vi "Deserialize Connections in Wrapper - Multiple Converter.vi"(11 "error in":errorcluster) -> (15 "error out":errorcluster)   [LabVIEW 2021, in "Converter.lvlib"]
uses:
  Converter.lvlib
  <vilib>/Utility/traverseref.llb/TRef TravTarget.ctl
  <vilib>/Utility/miscctls.llb/LVPointTypeDef.ctl
  <vilib>/Utility/traverseref.llb/VI Scripting - Traverse.lvlib
  Converter Reusables/Converter Reusables.lvlib
  Path Functions/Path Functions.lvlib
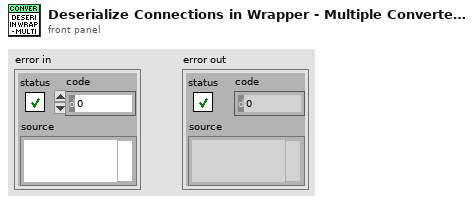
[diagram p1: front panel]
types:
  T1 = typedef "TRef TravTarget.ctl" = enum16{"FP", "BD", "Other"}
  T2 = typedef "LVPointTypeDef.ctl" = cluster{"Horizontal":i16, "Vertical":i16}
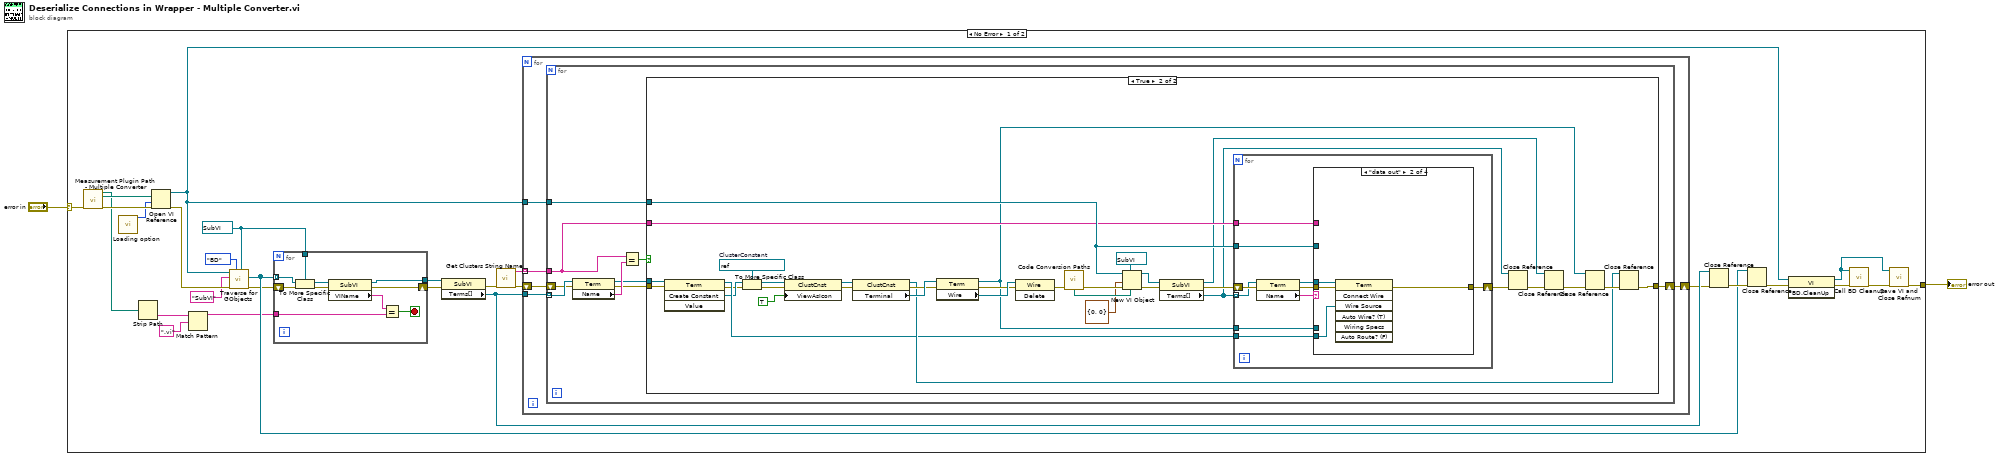
[diagram p0: block diagram]
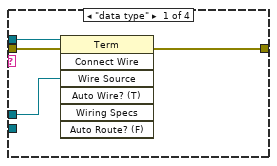
[diagram p3: hidden frame]
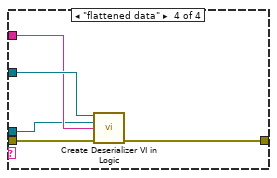
[diagram p5: hidden frame]
diagram:
  n1 = case shown="No Error" "error in" {
    selector: "error in" -> [w30 w114]
    tunnel: [w18 w114] -> w2
    frame No Error {
      w10 = refnum<vi> refnum ("Other Refnum")
      n2 = call "Measurement Plugin Path - Multiple Converter.vi"("error in"=w30) -> ("new code module"=w9:path, "wrapper path"=w29:path, "error out"=w28:errorcluster)  [unwired: 2 in, 10 out]
      n3 = call "Loading option.vi"() -> ("options"=w3:i32)  [unwired: 11 in]
      n4 = Strip Path(path=w9) -> (name=w8:string)  [unwired: 1 out]
      n5 = Open VI Reference(vi path=w29, options=w3, error in (no error)=w28) -> (vi reference=w17:refnum<vi>, error out=w27:errorcluster)  [unwired: 3 in]
      n6 = Match Pattern(string=w8, regular expression=".vi") -> (before substring=w6:string)  [unwired: 1 in, 3 out]
      n7 = call <vilib>:"Traverse for GObjects.vi"("Other Refnum"=w10, "Traverse Target"=TRef_TravTarget."BD", "error in (no error)"=w27, "Class Name"="SubVI", "VI Refnum"=w17) -> ("error out"=w11:errorcluster, "References"=w12:refnum<vi>[])  [unwired: 3 in, 2 out]
      n8 = for {
        tunnel: w12 -> [w112] mode=indexing
        tunnel: w10 -> [w111]
        tunnel: w6 -> [w106]
        shift-right: [w105] -> w5
        shift-left: w11 -> [w113]
        tunnel: [w104] -> w4
        stop <- w107 stop-if-true
        n9 = To More Specific Class(target class=w111, reference=w112, error in=w113) -> (specific class reference=w110:refnum<vi>, error out=w109:errorcluster)
        n10 = property class="SubVI"(reference=w110, error in=w109) -> (reference out=w104:refnum<vi>, error out=w105:errorcluster, "VIName"=w108:string)
        n11 = Equal?(x=w108, y=w106) -> (x = y?=w107:bool)
      }
      n12 = property class="SubVI"(reference=w4, error in=w5) -> (error out=w24:errorcluster, "Terms[]"=w21:refnum<vi>[])  [unwired: 1 out]
      n13 = call "Get Clusters String Name.vi"("error in"=w24) -> ("control names out"=w23:string[], "error out"=w22:errorcluster)  [unwired: 12 in, 1 out]
      n14 = for {
        tunnel: w21 -> [w35]
        tunnel: w23 -> [w33] mode=indexing
        shift-right: [w31] -> w20
        shift-left: w22 -> [w34]
        tunnel: w17 -> [w32]
        n15 = for {
          tunnel: w35 -> [w44] mode=indexing
          shift-right: [w37] -> w31
          shift-left: w34 -> [w42]
          tunnel: w33 -> [w36]
          tunnel: w32 -> [w38]
          n16 = property class="Term"(reference=w44, error in=w42) -> (reference out=w39:refnum<vi>, error out=w40:errorcluster, "Name"=w43:string)
          n17 = Equal?(x=w36, y=w43) -> (x = y?=w41:bool)
          n18 = case shown="True" w41 {
            tunnel: w40 -> [w45 w78]
            tunnel: w39 -> [_ w79]
            tunnel: w38 -> [_ w65]
            tunnel: [w45 w56] -> w37
            tunnel: w36 -> [_ w64]
            frame False {
            }
            frame True {
              w51 = refnum<vi> refnum  # ClusterConstant
              n19 = invoke class="Term" method="Create Constant"(reference=w79, error in=w78) -> (reference out=w55:refnum<vi>, error out=w49:errorcluster, "Create Constant"=w53:refnum<vi>)  [unwired: 2 in, 1 out]
              n20 = To More Specific Class(target class=w51, reference=w53, error in=w49) -> (specific class reference=w52:refnum<vi>, error out=w48:errorcluster)
              n21 = property class="ClustCnst"(reference=w52, error in=w48, "ViewAsIcon"=TRUE ("View As Icon")) -> (reference out=w47:refnum<vi>, error out=w46:errorcluster)
              n22 = property class="ClustCnst"(reference=w47, error in=w46) -> (reference out=w57:refnum<vi>, error out=w67:errorcluster, "Terminal"=w69:refnum<vi>)
              n23 = property class="Term"(reference=w69, error in=w67) -> (reference out=w54:refnum<vi>, error out=w66:errorcluster, "Wire"=w68:refnum<vi>)
              n24 = invoke class="Wire" method="Delete"(reference=w68, error in=w66) -> (error out=w77:errorcluster)  [unwired: 1 in, 2 out]
              n25 = call "Code Conversion Paths.vi"("error in"=w77) -> ("deserializer"=w76:path, "error out"=w75:errorcluster)  [unwired: 6 in, 7 out]
              n26 = New VI Object(vi object class=refnum<vi> refnum ("Other Refnum"), owner refnum=w65, position/next to=T2 {"Horizontal"=0, "Vertical"=0} ("location"), 6:w76, 8:w75) -> (object refnum=w72:refnum<vi>, 0:w71:errorcluster)  [unwired: 3 in]
              n27 = property class="SubVI"(reference=w72, error in=w71) -> (reference out=w60:refnum<vi>, error out=w70:errorcluster, "Terms[]"=w62:refnum<vi>[])
              n28 = for {
                tunnel: w62 -> [w86] mode=indexing
                shift-right: [w84] -> w63
                shift-left: w70 -> [w89]
                tunnel: w65 -> [w83]
                tunnel: w64 -> [w82]
                tunnel: w55 -> [w81]
                tunnel: w54 -> [w80]
                n29 = property class="Term"(reference=w86, error in=w89) -> (reference out=w85:refnum<vi>, error out=w88:errorcluster, "Name"=w87:string)
                n30 = case shown="\"data out\"" w87 {
                  tunnel: w88 -> [w92 w97 w98 w103]
                  tunnel: w85 -> [w93 w96 _ w100]
                  tunnel: [w91 w95 w98 w99] -> w84
                  tunnel: w83 -> [_ _ _ w102]
                  tunnel: w82 -> [_ _ _ w101]
                  tunnel: w81 -> [_ w94 _ _]
                  tunnel: w80 -> [w90 _ _ _]
                  frame "data type" {
                    n31 = invoke class="Term" method="Connect Wire"(reference=w93, error in=w92, "Wire Source"=w90) -> (error out=w91:errorcluster)  [unwired: 4 in, 6 out]
                  }
                  frame "data out" {
                    n32 = invoke class="Term" method="Connect Wire"(reference=w96, error in=w97, "Wire Source"=w94) -> (error out=w95:errorcluster)  [unwired: 4 in, 6 out]
                  }
                  frame Default {
                  }
                  frame "flattened data" {
                    n33 = call "Create Deserializer VI in Logic.vi"("vi refnum"=w102, "term refnum"=w100, "name"=w101, "error in"=w103) -> ("error out"=w99:errorcluster)  [unwired: 11 in]
                  }
                }
              }
              n34 = Close Reference(reference=w62, error in (no error)=w63) -> (error out=w61:errorcluster)
              n35 = Close Reference(reference=w60, error in (no error)=w61) -> (error out=w59:errorcluster)
              n36 = Close Reference(reference=w54, error in (no error)=w59) -> (error out=w58:errorcluster)
              n37 = Close Reference(reference=w57, error in (no error)=w58) -> (error out=w56:errorcluster)
            }
          }
        }
      }
      n38 = Close Reference(reference=w21, error in (no error)=w20) -> (error out=w19:errorcluster)
      n39 = Close Reference(reference=w12, error in (no error)=w19) -> (error out=w16:errorcluster)
      n40 = invoke class="VI" method="BD.CleanUp"(reference=w17, error in=w16) -> (reference out=w13:refnum<vi>, error out=w15:errorcluster)  [unwired: 1 in, 1 out]
      n41 = call "Call BD Cleanup.vi"("vi"=w13, "error in"=w15) -> ("error out"=w14:errorcluster)  [unwired: 13 in]
      n42 = call "Save VI and Close Refnum.vi"("vi refnum"=w13, "error in"=w14) -> ("error out"=w18:errorcluster)  [unwired: 13 in]
    }
    frame Error {
    }
  }
  "error out" <- w2
